vi "After TS Config Tasks.vi"(8 "error in":errorcluster, 11 "DeepU Test Stand in":refnum<class "DeepU Test Stand.lvclass">) -> (0 "error out":errorcluster, 3 "DeepU Test Stand out":refnum<class "DeepU Test Stand.lvclass">)   [LabVIEW 2019, in "Test Stands.lvlib" / "DeepU Test Stand.lvclass"]
uses:
  DeepU Test Stand.lvclass
  Generic Test Stand/TS Panel Method.ctl
  DeepU Test Stand.lvclass/DeepU Test Stand.ctl
  Generic Test Stand/Generic Test Stand.lvclass
  Results/DeepU Results/DeepU Results.lvclass
  Results/Results Method.ctl
  Results/Results.lvlib
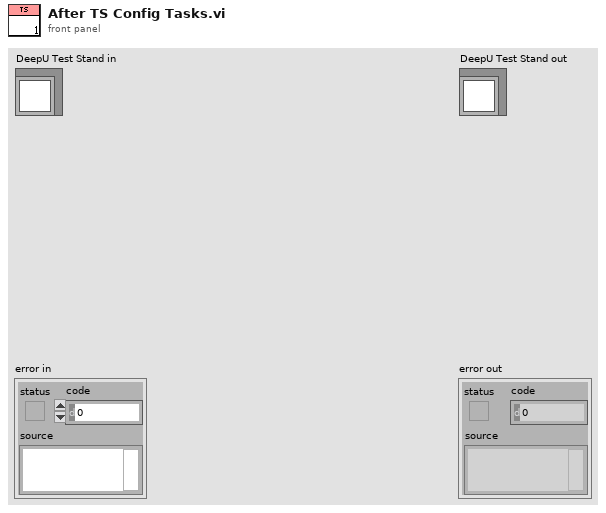
[diagram p1: front panel]
types:
  T1 = typedef "Results.lvlib/Results Method.ctl" = enum16{"Get", "Set"}
  T2 = typedef "Generic Test Stand.lvclass/TS Panel Method.ctl" = enum16{"Send to Panel", "Receive from Panel", "Update Panel View"}
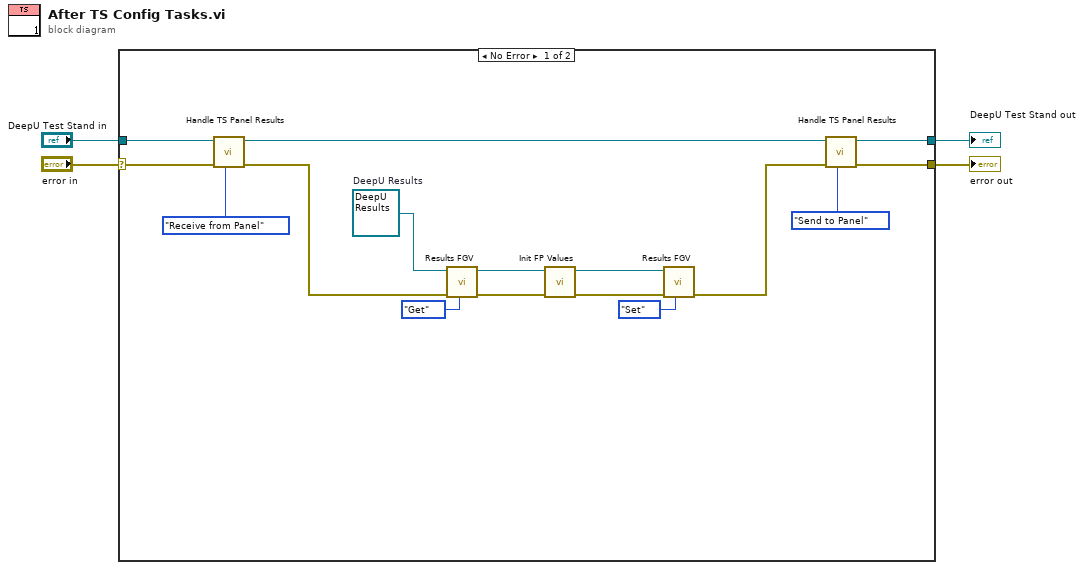
[diagram p0: block diagram]
diagram:
  n1 = case shown="No Error" "error in" {
    selector: "error in" -> [w15 w22]
    tunnel: [w14 w22] -> w4
    tunnel: [w19 w21] -> w3
    tunnel: "DeepU Test Stand in" -> [w20 w21]
    frame No Error {
      w13 = refnum<class "DeepU Results.lvclass"> refnum  # DeepU Results
      n2 = call-dynamic "Handle TS Panel Results.vi"("Method"=TS_Panel_Method."Receive from Panel", "error in"=w15, "DeepU Test Stand in"=w20) -> ("error out"=w6:errorcluster, "DeepU Test Stand out"=w16:refnum<class "DeepU Test Stand.lvclass">)  [unwired: 7 in]
      n3 = call-dynamic "Results FGV.vi"("Method"=Results_Method."Get", "error in"=w6, "DeepU Results in"=w13) -> ("error out"=w8:errorcluster, "DeepU Results out"=w10:refnum<class "DeepU Results.lvclass">)  [unwired: 7 in]
      n4 = call "Init FP Values.vi"("error in (no error)"=w8, "DeepU Results in"=w10) -> ("error out"=w7:errorcluster, "DeepU Results out"=w9:refnum<class "DeepU Results.lvclass">)  [unwired: 8 in]
      n5 = call-dynamic "Results FGV.vi"("Method"=Results_Method."Set", "error in"=w7, "DeepU Results in"=w9) -> ("error out"=w5:errorcluster)  [unwired: 7 in, 1 out]
      n6 = call-dynamic "Handle TS Panel Results.vi"("Method"=TS_Panel_Method."Send to Panel", "error in"=w5, "DeepU Test Stand in"=w16) -> ("error out"=w14:errorcluster, "DeepU Test Stand out"=w19:refnum<class "DeepU Test Stand.lvclass">)  [unwired: 7 in]
    }
    frame Error {
    }
  }
  "error out" <- w4
  "DeepU Test Stand out" <- w3
